vi "Error Test Channel Number.vi"(6 "indexing (0-based)":enum16{"0-based", "1-based"}(ring), 7 "reset (F)":bool, 8 "error in":errorcluster, 10 "channel #":u16, 11 "max channel number (31)":u16=31) -> (0 "error out":errorcluster)   [LabVIEW 2020]
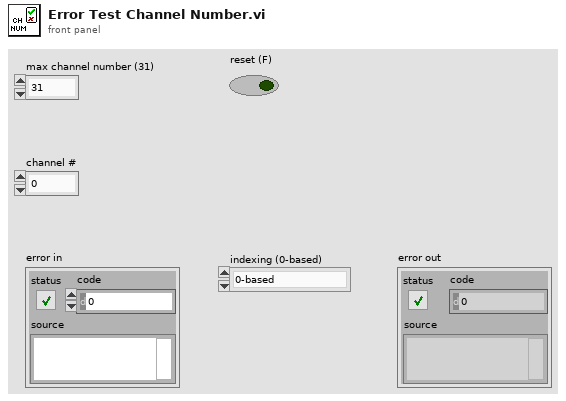
[diagram p1: front panel]
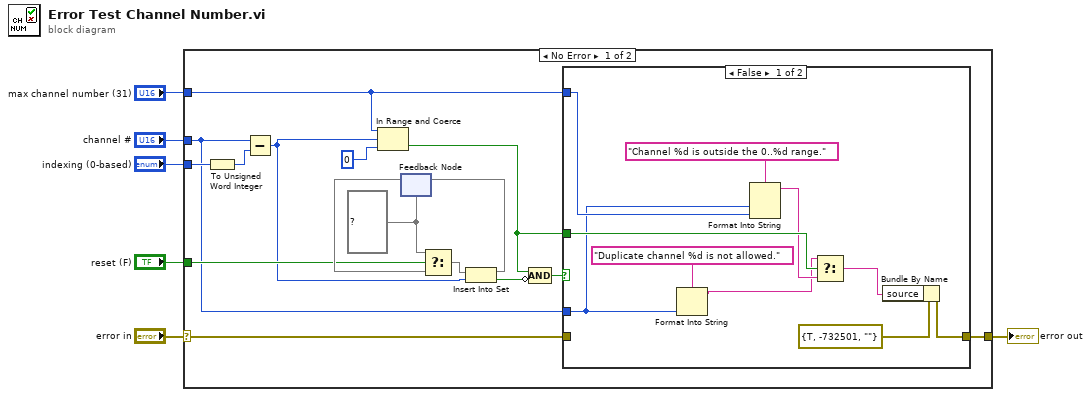
[diagram p0: block diagram]
diagram:
  n1 = case shown="No Error" "error in" {
    selector: "error in" -> [w22 w34]
    tunnel: [w21 w34] -> w5
    tunnel: "channel #" -> [w8 _]
    tunnel: "reset (F)" -> [w12 _]
    tunnel: "indexing (0-based)" -> [w10 _]
    tunnel: "max channel number (31)" -> [w7 _]
    frame No Error {
      w13 = set{u16} {} ("set in")
      n2 = To Unsigned Word Integer(number=w10) -> (unsigned 16bit integer=w9:u16)
      n3 = Subtract(x=w8, y=w9) -> (x-y=w11:u16)
      n4 = In Range and Coerce(upper limit=w7, x=w11, lower limit=u16 0 ("Channel #")) -> (In Range?=w16:bool)  [unwired: 1 out]
      n5 = feedback #1(w13) -> (w15:set{u16})
      n6 = Select(t=w13, s=w12, f=w15) -> (s? t:f=w14:set{u16})
      n7 = Insert Into Set(10:w11, 11:w14) -> (2:w18:bool, 3:w19:set{u16})
      n8 = feedback-in #1(w19) -> ()
      n9 = Compound Arithmetic op=AND(w16, invert w18) -> (w17:bool)
      n10 = case shown="False" w17 {
        tunnel: w22 -> [_ w33]
        tunnel: [w30 w33] -> w21
        tunnel: w8 -> [w23 _]
        tunnel: w16 -> [w31 _]
        tunnel: w7 -> [w27 _]
        frame False {
          n11 = Format Into String(format string="Duplicate channel %d is not allowed." ("source"), w23) -> (resulting string=w24:string)  [unwired: 2 in, 1 out]
          n12 = Format Into String(format string="Channel %d is outside the 0..%d range." ("source"), w23, w27) -> (resulting string=w28:string)  [unwired: 2 in, 1 out]
          n13 = Select(t=w24, s=w31, f=w28) -> (s? t:f=w26:string)
          n14 = Bundle By Name(cluster=errorcluster {"status"=TRUE, "code"=-732501, "source"=""} ("error constant"), "source"=w26) -> (w30:errorcluster)
        }
        frame True {
        }
      }
    }
    frame Error {
    }
  }
  "error out" <- w5
